vi "SeqEditor_init-EmptyTable.vi"(8 "error in (no error)":errorcluster, 11 "NLTest in":refnum<class "NLTest.lvclass">) -> (0 "error out":errorcluster, 3 "NLTest out":refnum<class "NLTest.lvclass">)   [LabVIEW 2017, in "NLTest.lvclass"]
uses:
  NLTest.lvclass
  NLTest.lvclass/NLTest.ctl
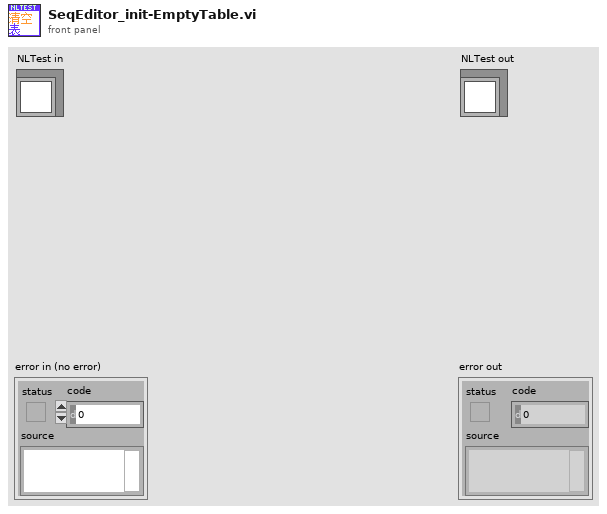
[diagram p1: front panel]
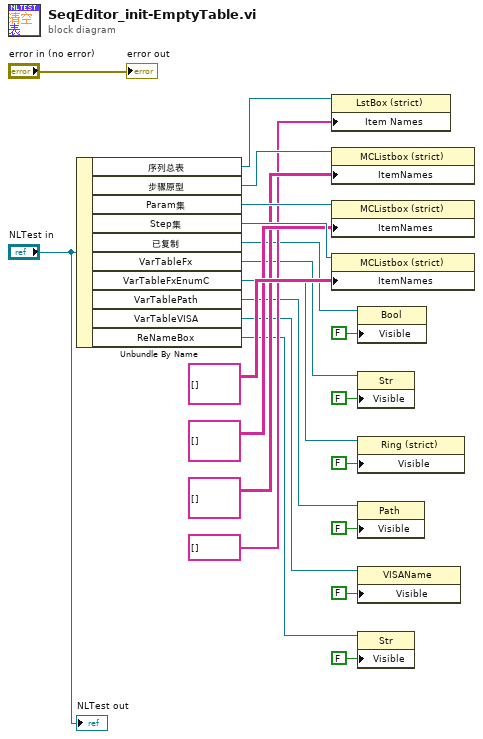
[diagram p0: block diagram]
diagram:
  n1 = Unbundle By Name("NLTest in") -> ("序列总表"=w20:refnum<vi>, "步骤原型"=w19:refnum<vi>, "Param集"=w18:refnum<vi>, "Step集"=w17:refnum<vi>, "已复制"=w12:refnum<vi>, "VarTableFx"=w9:refnum<vi>, "VarTableFxEnumC"=w7:refnum<vi>, "VarTablePath"=w5:refnum<vi>, "VarTableVISA"=w3:refnum<vi>, "ReNameBox"=w1:refnum<vi>)
  n2 = property class="LstBox (strict)"(reference=w20, "Item Names"=string[] []) -> ()  [unwired: 1 in, 2 out]
  n3 = property class="MCListbox (strict)"(reference=w19, "ItemNames"=string[][] [] ("Item Names")) -> ()  [unwired: 1 in, 2 out]
  n4 = property class="MCListbox (strict)"(reference=w18, "ItemNames"=string[][] [] ("Item Names")) -> ()  [unwired: 1 in, 2 out]
  n5 = property class="MCListbox (strict)"(reference=w17, "ItemNames"=string[][] [] ("Item Names")) -> ()  [unwired: 1 in, 2 out]
  n6 = property class="Bool"(reference=w12, "Visible"=FALSE) -> ()  [unwired: 1 in, 2 out]
  n7 = property class="Str"(reference=w9, "Visible"=FALSE) -> ()  [unwired: 1 in, 2 out]
  n8 = property class="Ring (strict)"(reference=w7, "Visible"=FALSE) -> ()  [unwired: 1 in, 2 out]
  n9 = property class="Path"(reference=w5, "Visible"=FALSE) -> ()  [unwired: 1 in, 2 out]
  n10 = property class="VISAName"(reference=w3, "Visible"=FALSE) -> ()  [unwired: 1 in, 2 out]
  n11 = property class="Str"(reference=w1, "Visible"=FALSE) -> ()  [unwired: 1 in, 2 out]
  "error out" <- "error in (no error)"
  "NLTest out" <- "NLTest in"
